vi "Create Python TCP Server.vi"(7 "net address (0: Listen on All Adaptors)":u32, 8 "error in (no error)":errorcluster, 9 "max connections (0: no limit)":u32, 10 "TCP port":u16) -> (0 "error out":errorcluster, 2 "Python Method Call":refnum<user-event>, 3 "TCP Server Refnum":refnum<class "JKI TCP Server.lvclass">)   [LabVIEW 2020, in "jki_python_bridge.lvlib" / "Server.lvclass"]
uses:
  Server.lvclass
  Server.lvclass/Server.ctl
  Python TCP Connection Handler.vi
  Call/Call.lvclass
  <vilib>/addons/_JKI.lib/_JKI_lib_TCP_Server.llb/JKI TCP Server.lvclass
panel:
  # "Copyright © 2004-2008 JKI. All rights reserved.\n\nAuthor: Jim Kring [jim.kring@jameskring.com]\n\nThis library is provided \"AS IS\" ,WITHOUT WARRANTIES OR \nCONDITIONS OF ANY KIND, either express or implied.\n\nJames Kring, Inc. -- http://www.jameskring.com"
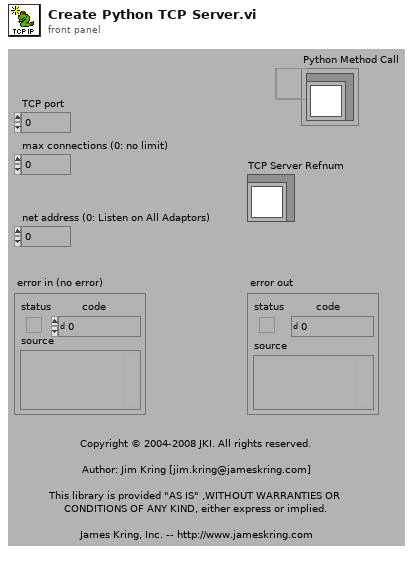
[diagram p1: front panel]
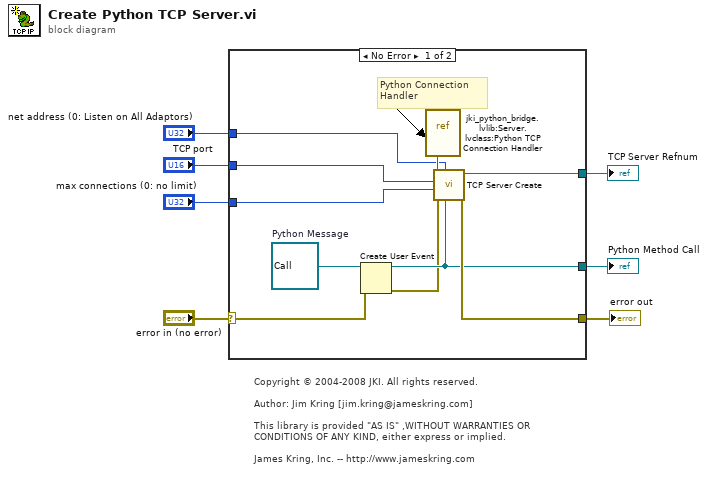
[diagram p0: block diagram]
diagram:
  # "Copyright © 2004-2008 JKI. All rights reserved.\n\nAuthor: Jim Kring [jim.kring@jameskring.com]\n\nThis library is provided \"AS IS\" ,WITHOUT WARRANTIES OR \nCONDITIONS OF ANY KIND, either express or implied.\n\nJames Kring, Inc. -- http://www.jameskring.com"
  n1 = case shown="No Error" "error in (no error)" {
    selector: "error in (no error)" -> [w12 w18]
    tunnel: [w16 w18] -> w4
    tunnel: [w15 _] -> w5
    tunnel: [w14 _] -> w6
    tunnel: "max connections (0: no limit)" -> [w11 _]
    tunnel: "TCP port" -> [w10 _]
    tunnel: "net address (0: Listen on All Adaptors)" -> [w9 _]
    frame No Error {
      w8 = refnum<class "Call.lvclass"> refnum  # Python Message
      # "Python Connection \nHandler"
      n2 = Create User Event(user event datatype=w8, error in=w12) -> (user event=w14:refnum<user-event>, error out=w13:errorcluster)
      n3 = vi-ref "jki_python_bridge.lvlib:Server.lvclass:Python TCP Connection Handler.vi"() -> ("vi reference"=w17:refnum<vi>)
      n4 = call <vilib>:"TCP Server Create.vi"("Additional Data"=w14, "net address (0: Listen on All Adaptors)"=w9, "error in (no error)"=w13, "max connections (0: no limit)"=w11, "port"=w10, "Connection Handler Call-Back VI RefNum"=w17) -> ("error out"=w16:errorcluster, "TCP Server"=w15:refnum<class "JKI TCP Server.lvclass">)  [unwired: 4 in]
    }
    frame Error {
    }
  }
  "Python Method Call" <- w6
  "TCP Server Refnum" <- w5
  "error out" <- w4
